vi "IsContainsDuplicateCtrlNames.vi"(0 "VI Reference In":refnum<vi>, 11 "Error In":errorcluster) -> (4 "VI Reference Out":refnum<vi>, 6 "Duplicate Found?":bool, 15 "Error Out":errorcluster)   [LabVIEW 2019, in "Drona.lvlib"]
doc: "This VI return true if it contains duplicate control labels"
uses:
  Drona.lvlib
  79b6dddf-13ba-456f-a10f-6c608e784c74.vi
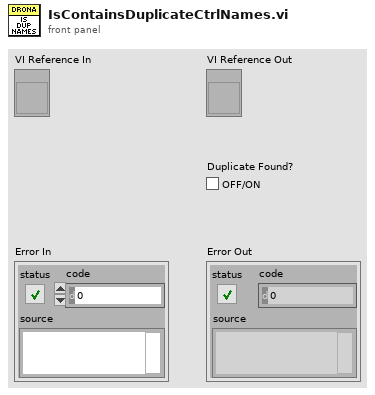
[diagram p1: front panel]
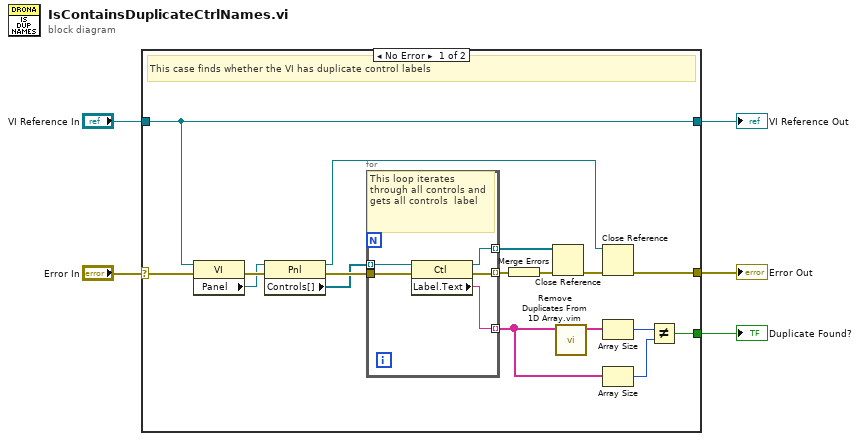
[diagram p0: block diagram]
diagram:
  n1 = case shown="No Error" "Error In" {
    selector: "Error In" -> [w22 w29]
    tunnel: "VI Reference In" -> [w14 w28]
    tunnel: [w14 w28] -> w3
    tunnel: [w6 w29] -> w2
    tunnel: [w9 _] -> w1
    frame No Error {
      # "This case finds whether the VI has duplicate control labels"
      n2 = property class="VI"(reference=w14, error in=w22) -> (error out=w21:errorcluster, "Panel"=w20:refnum<vi>)  [unwired: 1 out]
      n3 = property class="Pnl"(reference=w20, error in=w21) -> (reference out=w8:refnum<vi>, error out=w19:errorcluster, "Controls[]"=w18:refnum<vi>[])
      n4 = for {
        tunnel: w19 -> [w27]
        tunnel: [w26] -> w17 mode=indexing
        tunnel: w18 -> [w25] mode=indexing
        tunnel: [w24] -> w15 mode=indexing
        tunnel: [w23] -> w13 mode=indexing
        # "This loop iterates through all controls and gets all controls  label"
        n5 = property class="Ctl"(reference=w25, error in=w27) -> (reference out=w24:refnum<vi>, error out=w26:errorcluster, "Label.Text"=w23:string)
      }
      n6 = Merge Errors(w17) -> (w16:errorcluster)
      n7 = Close Reference(reference=w15, error in (no error)=w16) -> (error out=w7:errorcluster)
      n8 = call "Remove Duplicates From 1D Array.vim"("array"=w13) -> ("array with duplicates removed"=w12:string[])  [unwired: 10 in]
      n9 = Close Reference(reference=w8, error in (no error)=w7) -> (error out=w6:errorcluster)
      n10 = Array Size(array=w12) -> (size(s)=w10:i32)
      n11 = Array Size(array=w13) -> (size(s)=w11:i32)
      n12 = Not Equal?(x=w10, y=w11) -> (x != y?=w9:bool)
    }
    frame Error {
      # "If error, this case pass that error message only"
    }
  }
  "Error Out" <- w2
  "VI Reference Out" <- w3
  "Duplicate Found?" <- w1
